vi "CopyUserEventstoRunIDFolder.vi"(11 "Data Cluster in":T1) -> (3 "Data Cluster out":T1)   [LabVIEW 2026, in "Core.lvlib"]
uses:
  Core.lvlib
  Module Data--cluster.ctl
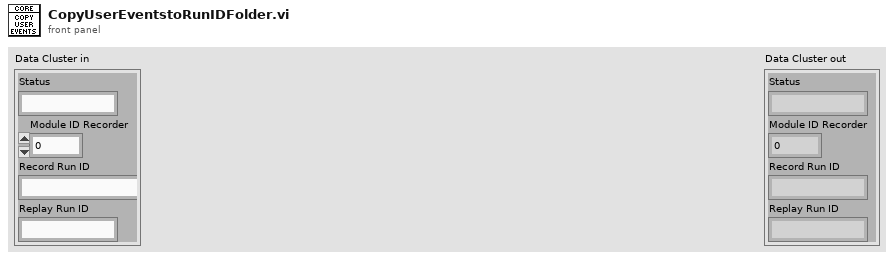
[diagram p1: front panel]
types:
  T1 = typedef "Core.lvlib/Module Data--cluster.ctl" = cluster{"Status":string, "Module ID Recorder":i32, "Record Run ID":string, "Replay Run ID":string}
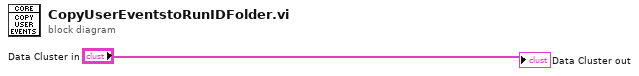
[diagram p0: block diagram]
diagram:
  "Data Cluster out" <- "Data Cluster in"
